vi "close.vi"(8 "error in":errorcluster, 11 "Doc in":refnum<class "Doc.lvclass">) -> (0 "error out":errorcluster)   [LabVIEW 2020, in "toml_edit.lvlib" / "Doc.lvclass"]
uses:
  Doc.lvclass
  Doc.lvclass/Doc.ctl
  dragon_toml_64.dll
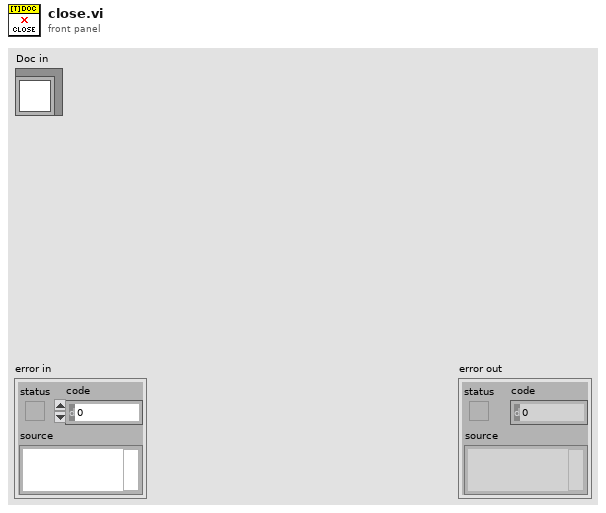
[diagram p1: front panel]
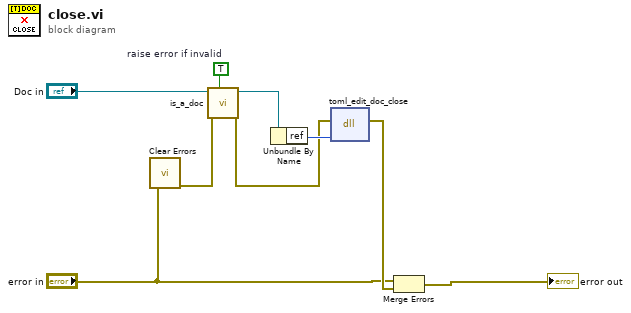
[diagram p0: block diagram]
diagram:
  w6 = TRUE  # raise error if invalid
  n1 = call <vilib>:"Clear Errors.vi"("error in (no error)"="error in") -> ("error out"=w3:errorcluster)  [unwired: 5 in, 1 out]
  n2 = call "is_a_doc.vi"("raise error if invalid? (False)"=w6, "error in (no error)"=w3, "Doc in"="Doc in") -> ("error out"=w2:errorcluster, "Doc out"=w7:refnum<class "Doc.lvclass">)  [unwired: 6 in, 1 out]
  n3 = Unbundle By Name(w7) -> ("ref"=w4:u64)
  n4 = dll-call lib="C:/projects/dragon-desktop/source/submodules/toml-edit-labview/lv_src/dragon_toml_*.dll" fn="toml_edit_doc_close"(error in=w2, "ptr"=w4) -> (error out=w5:errorcluster)  [unwired: 4 in, 1 out]
  n5 = Merge Errors("error in", w5) -> (→"error out":errorcluster)
